vi "Enqueue Data.vi"(8 "error in":errorcluster, 10 "UI GUID":string, 11 "Data":string[][](array[string])) -> (0 "error out":errorcluster, 3 "overflow?":bool)   [LabVIEW 2025, in "CAN-LIN Raw Bus Capture UI.lvlib"]
uses:
  CAN-LIN Raw Bus Capture UI.lvlib
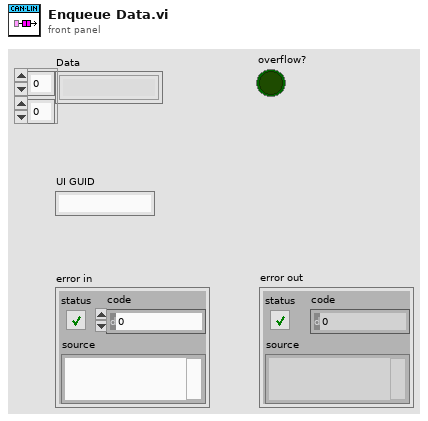
[diagram p1: front panel]
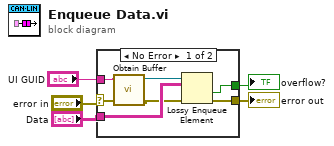
[diagram p0: block diagram]
diagram:
  n1 = case shown="No Error" "error in" {
    selector: "error in" -> [w8 w13]
    tunnel: [w12 w13] -> w3
    tunnel: "Data" -> [w11 _]
    tunnel: [w10 _] -> w2
    tunnel: "UI GUID" -> [w6 _]
    frame No Error {
      n2 = call "Obtain Buffer.vi"("error in (no error)"=w8, "UI GUID"=w6) -> ("error out"=w9:errorcluster, "Table Queue"=w7:refnum<queue>)  [unwired: 8 in]
      n3 = Lossy Enqueue Element(queue=w7, element=w11, error in (no error)=w9) -> (overflow?=w10:bool, error out=w12:errorcluster)  [unwired: 2 out]
    }
    frame Error {
    }
  }
  "error out" <- w3
  "overflow?" <- w2
